vi "ZM-CI-handlePackage.vi"(8 "error in (no error)":errorcluster, 10 "package":refnum<class "ZM-PC-package.lvclass">, 11 "ZM-CI-package_handler in":refnum<class "ZM-CI-package_handler.lvclass">) -> (0 "error out":errorcluster, 3 "ZM-CI-package_handler out":refnum<class "ZM-CI-package_handler.lvclass">)   [LabVIEW 2020, in "ZM-CI-common_interfaces.lvlib" / "ZM-CI-package_handler.lvclass"]
doc: "Interface method: delivers one package to the actor that implements ZM-CI-package_handler. No logic here; each actor's override decides."
uses:
  ZM-CI-package_handler.lvclass
  ZM-PC-packages/ZM-PC-package/ZM-PC-package.lvclass
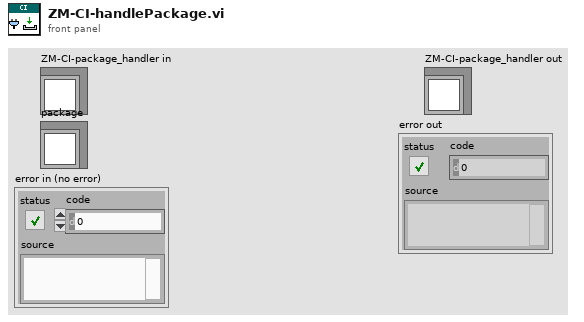
[diagram p1: front panel]
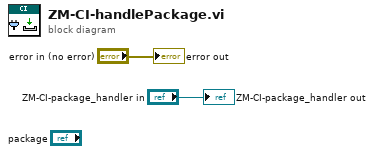
[diagram p0: block diagram]
diagram:
  "ZM-CI-package_handler out" <- "ZM-CI-package_handler in"
  "error out" <- "error in (no error)"
